vi "YAV_Alarm_Output.vi"(0 "DO0":bool, 1 "DO1":bool, 2 "错误输入（无错误）":errorcluster, 3 "ID":u32 format="%.0x", 7 "Hardware Enable":bool) -> (4 "错误输出":errorcluster, 5 "ID 2":u32 format="%.0x", 6 "Encoded Buffer":dbl[](array[numeric]))   [LabVIEW 2020]
doc: "PLACEHOLDER: error interface only. Alarm simulation NOT implemented."
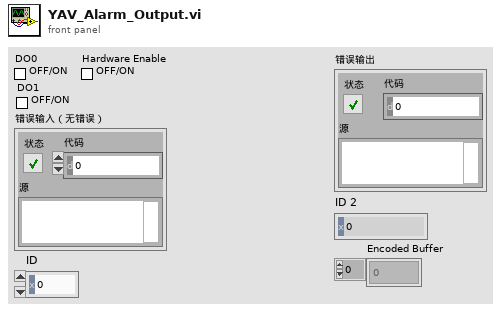
[diagram p1: front panel]
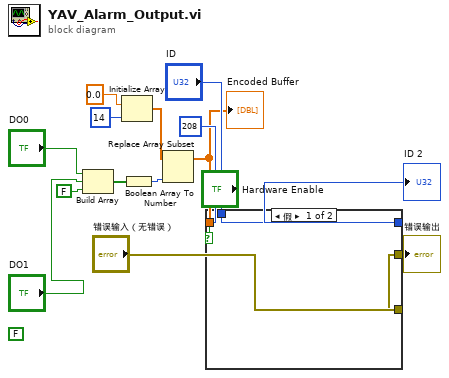
[diagram p0: block diagram]
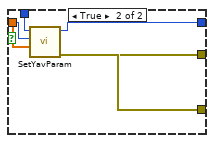
[diagram p2: hidden frame]
diagram:
  (unwired) FALSE
  n1 = Build Array("DO0", "DO1", FALSE ("元素")) -> (w10:bool[])
  n2 = Initialize Array(0.0 ("元素"), 14 ("维数大小")) -> (w14:dbl[])
  n3 = Boolean Array To Number(Boolean array=w10) -> (number=w15:u32)
  n4 = Replace Array Subset(array=w14, new element=w15) -> (w4:dbl[])  [unwired: 1 in]
  "Encoded Buffer" <- w4
  n5 = case shown="假" "Hardware Enable" {
    tunnel: "错误输入（无错误）" -> [w16 w23]
    tunnel: u8 208 ("CMD") -> [_ w22]
    tunnel: "ID" -> [w17 w21]
    tunnel: [w16 w20] -> w6
    tunnel: [w17 w19] -> w5
    tunnel: w4 -> [_ w18]
    frame False {
    }
    frame True {
      n6 = call "SetYavParam.vi"("错误输入（无错误）"=w23, "WriteParam"=w18, "CMD"=w22, "ID"=w21) -> ("错误输出"=w20:errorcluster, "ID"=w19:u32)  [unwired: 6 in]
    }
  }
  "错误输出" <- w6
  "ID 2" <- w5
